vi "VIH - CHM Project - HHP Support - Parse Window Properties.vi"(11 "Window property":string) -> (3 "Properties":string[](array[string]))   [LabVIEW 2014]
doc: "::: VI Helpeks :::\nCopyright (c) 2000-2026 Konstantin Shifershteyn. All rights reserved."
panel:
  # "VI Helpeks\nCopyright (c) 2012-2026 Konstantin Shifershteyn"
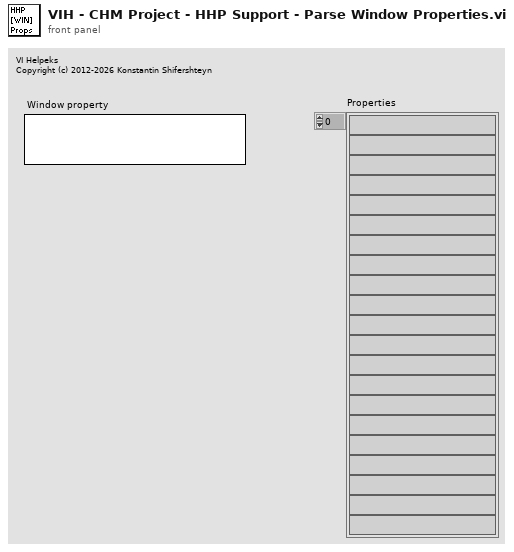
[diagram p1: front panel]
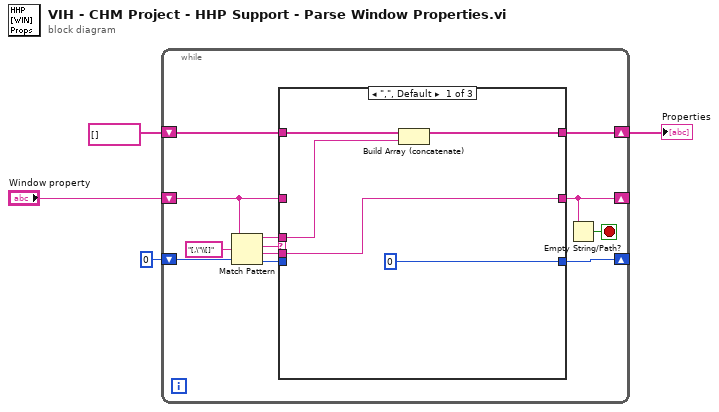
[diagram p0: block diagram]
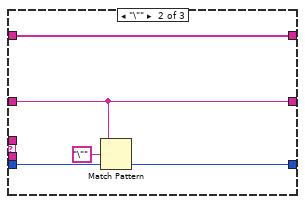
[diagram p2: hidden frame]
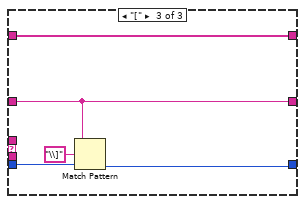
[diagram p3: hidden frame]
diagram:
  n1 = while {
    shift-right: [w6] -> _
    shift-left: "Window property" -> [w5]
    shift-right: [w12] -> w3
    shift-left: string[] [] -> [w14]
    shift-right: [w9] -> _
    shift-left: 0 ("offset past match") -> [w10]
    stop <- w7 stop-if-true
    n2 = Match Pattern(string=w5, regular expression="[,\"\\[]", offset (0)=w10) -> (before substring=w13:string, match substring=w15:string, after substring=w11:string, offset past match=w8:i32)
    n3 = case shown="\",\", Default" w15 {
      tunnel: w14 -> [w21 w26 w31]
      tunnel: w13 -> [w20 _ _]
      tunnel: [w19 w26 w31] -> w12
      tunnel: [w18 w24 w30] -> w6
      tunnel: w11 -> [w18 _ _]
      tunnel: [0 ("offset past match") w23 w28] -> w9
      tunnel: w8 -> [_ w25 w29]
      tunnel: w5 -> [_ w24 w30]
      frame ",", Default {
        n4 = Build Array (concatenate)(w21, w20) -> (w19:string[])
      }
      frame "\"" {
        n5 = Match Pattern(string=w24, regular expression="\"", offset (0)=w25) -> (offset past match=w23:i32)  [unwired: 3 out]
      }
      frame "[" {
        n6 = Match Pattern(string=w30, regular expression="\\]", offset (0)=w29) -> (offset past match=w28:i32)  [unwired: 3 out]
      }
    }
    n7 = Empty String/Path?(string/path=w6) -> (empty?=w7:bool)
  }
  "Properties" <- w3
